vi "CSM - Mark All Temp Variables as Permanent.vi"(8 "error in (no error)":errorcluster, 9 "Path (\"\" to Use Default File)":path) -> (2 "error out":errorcluster)   [LabVIEW 2017, in "INI-Static-Variable-Support.lvlib"]
doc: "Marks all temporary variables as permanent variables and stores the variables into the specified configuration file.\n\n<b>Note</b>: Although marked as permanent variables, these variables will still not be synchronized to the file if CSM - Sync Configuration Variables to File VI is not used.\n\n\n> [!NOTE] <b>CSM INI-Variable Configuration File Path</b>\n>\n> - <b>Development State</b>: The first INI configuration file found in the Application Directory. If no configuration file exists, it defaults to `csm-app.ini`.\n> - <b>Post-Compilation</b>: An INI configuration file in the same directory as the executable file, with the same name as the executable. LabVIEW automatically generates this file after compilation.\n> - Supports loading multiple configuration files. Configuration items in files loaded later will overwrite identical items in previously loaded files.\n> - Configuration files can use the `[__include]` section to reference other configuration files.\n> - Supports both relative and absolute paths.\n> - Relative paths are relative to the path of the current configuration file.\n> - The name of the configuration file in the `[__include]` section is not critical, as long as the path is correct.\n> - To avoid circular references, the same configuration file will be automatically ignored if loaded a second time.\n\n\n-- <b>Controls</b> --\n- <b>Path (\"\" to Use Default File)</b>: Configuration file path. An empty string indicates the default INI file."
uses:
  INI-Static-Variable-Support.lvlib
  _Support/_fgv-oper.ctl
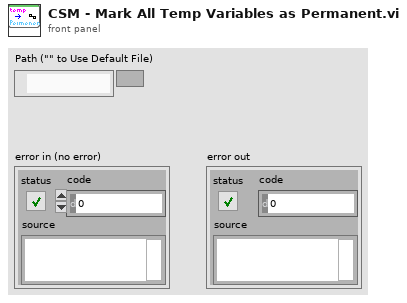
[diagram p1: front panel]
types:
  T1 = typedef "INI-Static-Variable-Support.lvlib/_fgv-oper.ctl" = enum16{"Read", "Write", "Sync", "Sessions", "List Keys", "Load", "List Files", "List Variables", "List Permanent Variables", "Mark Temp Variable as Permenent", "unload", "INIConfig(Memory)", "Reset", "Restore Variable Value"}
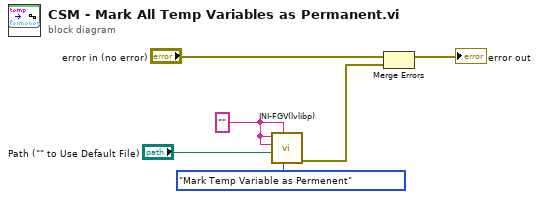
[diagram p0: block diagram]
diagram:
  w1 = "" (">> Variable Name >>")
  n1 = call "INI-FGV(lvlibp).vi"("Enum"=_fgv-oper."Mark Temp Variable as Permenent", "Prefered Section"=w1, "Path"="Path (\"\" to Use Default File)", ">> Default Value >>"=w1, ">> Variable Name >>"=w1) -> ("error out"=w4:errorcluster)  [unwired: 3 in, 3 out]
  n2 = Merge Errors("error in (no error)", w4) -> (→"error out":errorcluster)
